vi "GetApplicationSettings.vi"(0 "Application in":refnum<class "Application.lvclass">, 5 "error in (no error)":errorcluster) -> (14 "Application out":refnum<class "Application.lvclass">, 19 "error out":errorcluster)   [LabVIEW 2019, in "Application.lvclass"]
uses:
  Application.lvclass
  Application.lvclass/Application.ctl
  RobotType.ctl
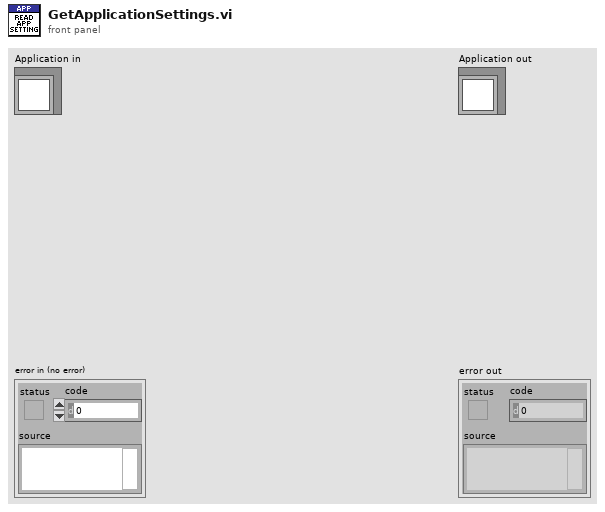
[diagram p1: front panel]
types:
  T1 = typedef "Application.lvclass/RobotType.ctl" = enum16{"UR E-Series", "UR CB-Series"}
  T2 = typedef "NI_LVConfig.lvlib/Config Data RefNum.ctl" = refnum<k1>
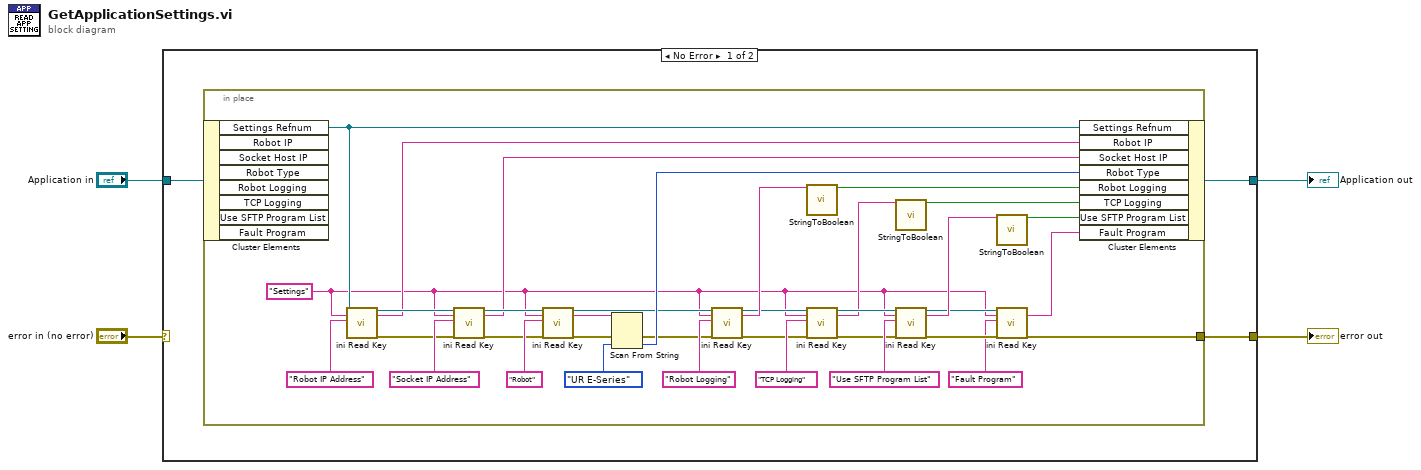
[diagram p0: block diagram]
diagram:
  n1 = case shown="No Error" "error in (no error)" {
    selector: "error in (no error)" -> [_ w44]
    tunnel: [w5 w44] -> w3
    tunnel: [w6 w43] -> w1
    tunnel: "Application in" -> [w7 w43]
    frame No Error {
      n2 = in-place {
        in-place-border: [w9] -> w5
        w11 = "Settings" ("Section")
        n3 = in-place-cluster #1(w7) -> ("Settings Refnum"=w42:T2)  [unwired: 7 out]
        n4 = call "ini Read Key.vi"("Refnum in"=w42, "Section"=w11, "Key"="Robot IP Address") -> ("Refnum out"=w35:T2, "value"=w29:string, "error out"=w30:errorcluster)  [unwired: 14 in]
        n5 = call "ini Read Key.vi"("Refnum in"=w35, "Section"=w11, "Key"="Socket IP Address", "Error In"=w30) -> ("Refnum out"=w34:T2, "value"=w31:string, "error out"=w33:errorcluster)  [unwired: 13 in]
        n6 = call "ini Read Key.vi"("Refnum in"=w34, "Section"=w11, "Key"="Robot", "Error In"=w33) -> ("Refnum out"=w24:T2, "value"=w36:string, "error out"=w39:errorcluster)  [unwired: 13 in]
        n7 = Scan From String(input string=w36, error in=w39, default 1=RobotType."UR E-Series" ("RobotType")) -> (error out=w23:errorcluster, output 1=w37:T1)  [unwired: 2 in, 2 out]
        n8 = call "ini Read Key.vi"("Refnum in"=w24, "Section"=w11, "Key"="Robot Logging", "Error In"=w23) -> ("Refnum out"=w19:T2, "value"=w21:string, "error out"=w18:errorcluster)  [unwired: 13 in]
        n9 = call "StringToBoolean.vi"("String"=w21) -> ("Boolean"=w22:bool)  [unwired: 17 in, 1 out]
        n10 = call "ini Read Key.vi"("Refnum in"=w19, "Section"=w11, "Key"="TCP Logging", "Error In"=w18) -> ("Refnum out"=w16:T2, "value"=w15:string, "error out"=w14:errorcluster)  [unwired: 13 in]
        n11 = call "StringToBoolean.vi"("String"=w15) -> ("Boolean"=w17:bool)  [unwired: 17 in, 1 out]
        n12 = call "ini Read Key.vi"("Refnum in"=w16, "Section"=w11, "Key"="Use SFTP Program List", "Error In"=w14) -> ("Refnum out"=w12:T2, "value"=w27:string, "error out"=w13:errorcluster)  [unwired: 13 in]
        n13 = call "StringToBoolean.vi"("String"=w27) -> ("Boolean"=w26:bool)  [unwired: 17 in, 1 out]
        n14 = call "ini Read Key.vi"("Refnum in"=w12, "Section"=w11, "Key"="Fault Program", "Error In"=w13) -> ("value"=w8:string, "error out"=w9:errorcluster)  [unwired: 13 in, 1 out]
        n15 = in-place-cluster #1("Settings Refnum"=w42, "Robot IP"=w29, "Socket Host IP"=w31, "Robot Type"=w37, "Robot Logging"=w22, "TCP Logging"=w17, "Use SFTP Program List"=w26, "Fault Program"=w8) -> (w6:refnum<class "Application.lvclass">)
      }
    }
    frame Error {
    }
  }
  "error out" <- w3
  "Application out" <- w1
